vi "FuncVI-AutoCorrel.vi"(5 "InstanceRef":T2, 9 "arg list":T1[](array[typedef]) {"num" format="%.2f"}) -> (0 "error out":bool, 3 "result":T1 {"num" format="%.2f"})   [LabVIEW 2021]
doc: "::: CalcExpress Toolkit :::\nCopyright (c) 2000-2026 Konstantin Shifershteyn. All rights reserved."
uses:
  cetypes.llb/CalcExpress Function Argument Info.ctl
  cetypes.llb/CalcExpress Instance RefNum.ctl
  <vilib>/Analysis/2dsp.llb/1D Auto Correlation (DBL).vi
  <vilib>/Analysis/NI_AALPro.lvlib
panel:
  in  "max arg num":i32=1
  in  "min arg num":i32=1
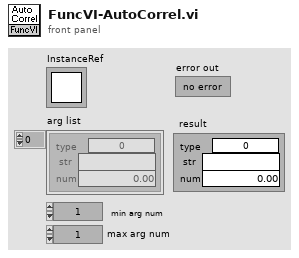
[diagram p1: front panel]
types:
  T1 = typedef "CalcExpress Function Argument Info.ctl" = cluster{"type":u32, "str":string, "num":dbl}
  T2 = typedef "CalcExpress Instance RefNum.ctl" = refnum<k1>
  T3 = enum8{"String", "DBL Number", "identifier", "1D Array of DBL", "2D Array of DBL", "CDB Number", "1D Array of CDB", "2D Array of CDB", "1D Array of String", "2D Array of String", "Unknown data type"}
  T4 = cluster{"index":i32, "type":enum8{"String", "DBL Number", "identifier", "1D Array of DBL", "2D Array of DBL", "CDB Number", "1D Array of CDB", "2D Array of CDB", "Unknown data type"}, "default num":dbl, "default str":string}[]
  T5 = cluster{"type":enum8{"String", "DBL Number", "identifier", "1D Array of DBL", "2D Array of DBL", "CDB Number", "1D Array of CDB", "2D Array of CDB", "1D Array of String", "2D Array of String", "Unknown data type"}, "data string":string, dbl}
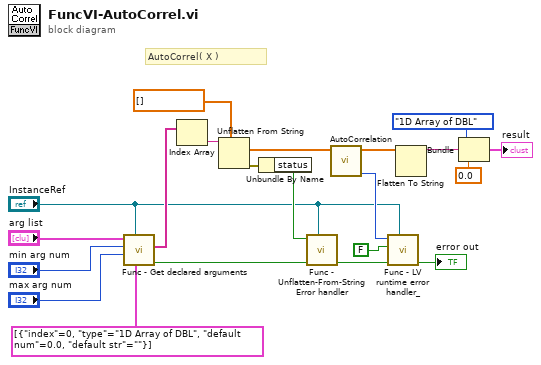
[diagram p0: block diagram]
diagram:
  # "AutoCorrel( X )"
  n1 = call "Func - Get declared arguments.vi"("arg descriptors"=T4 [{"index"=0, "type"=enum."1D Array of DBL", "default num"=0.0, "default str"=""}] ("args descriptors"), "InstanceRef"="InstanceRef", "max arg num"="max arg num", "min arg num"="min arg num", "arg list"="arg list") -> ("error out"=w8:bool, "str list"=w18:string[])  [unwired: 3 in, 2 out]
  n2 = Index Array(array=w18) -> (element=w17:string)  [unwired: 1 in]
  n3 = Unflatten From String(type=dbl[] [], binary string=w17) -> (value=w15:dbl[], error out=w1:errorcluster)  [unwired: 3 in, 1 out]
  n4 = Unbundle By Name(w1) -> ("status"=w7:bool)
  n5 = call "Func - Unflatten-From-String Error handler.vi"("InstanceRef"="InstanceRef", "error in"=w8, "Unflatten Error status"=w7) -> ("error out"=w6:bool)  [unwired: 6 in]
  n6 = call-poly <vilib>:"AutoCorrelation.vi"("X"=w15) -> ("error"=w10:i32, "Rxx"=w14:dbl[])  [unwired: 9 in]
  n7 = call "Func - LV runtime error handler_.vi"("InstanceRef"="InstanceRef", "error in"=w6, "Gen CE error?"=FALSE, "LabVIEW error code"=w10) -> ("error out"=→"error out":bool)  [unwired: 7 in]
  n8 = Flatten To String(anything=w14) -> (data string=w12:string)  [unwired: 3 in, 2 out]
  n9 = Bundle("type"=T3."1D Array of DBL", "data string"=w12, 0.0) -> (→"result":T5)  [unwired: 1 in]
